vi "KeyboardSimulationCore.vi"(0 "Key Array":T3(array[cluster]) {"Key" items=["LBUTTON"=1, "RBUTTON"=2, "CANCEL"=3, "MBUTTON"=4, "BACKSPACE"=8, "TAB"=9, "CLEAR"=12, "ENTER"=13, "SHIFT"=16, "CTRL"=17, "ALT"=18, "PAUSE"=19, "CAPITAL"=20, "ESCAPE"=27, "SPACE"=32, "PAGEUP"=33, "PAGEDOWN"=34, "END"=35, "HOME"=36, "LEFTARROW"=37, "UPARROW"=38, "RIGHTARROW"=39, "DOWNARROW"=40, "SELECT"=41, "PRINT"=42, "EXECUTE"=43, "PRINTSCREEN"=44, "INSERT"=45, "DELETE"=46, "HELP"=47, "0"=48, "1"=49, "2"=50, "3"=51, "4"=52, "5"=53, "6"=54, "7"=55, "8"=56, "9"=57, "A"=65, "B"=66, "C"=67, "D"=68, "E"=69, "F"=70, "G"=71, "H"=72, "I"=73, "J"=74, "K"=75, "L"=76, "M"=77, "N"=78, "O"=79, "P"=80, "Q"=81, "R"=82, "S"=83, "T"=84, "U"=85, "V"=86, "W"=87, "X"=88, "Y"=89, "Z"=90, "LWIN"=91, "RWIN"=92, "APPS"=93, "NUMPAD0"=96, "NUMPAD1"=97, "NUMPAD2"=98, "NUMPAD3"=99, "NUMPAD4"=100, "NUMPAD5"=101, "NUMPAD6"=102, "NUMPAD7"=103, "NUMPAD8"=104, "NUMPAD9"=105, "MULTIPLY"=106, "ADD"=107, "SEPERATOR"=108, "SUBTRACT"=109, "DECIMAL"=110, "DIVIDE"=111, "F1"=112, "F2"=113, "F3"=114, "F4"=115, "F5"=116, "F6"=117, "F7"=118, "F8"=119, "F9"=120, "F10"=121, "F11"=122, "F12"=123, "F13"=124, "F14"=125, "F15"=126, "F16"=127, "F17"=128, "F18"=129, "F19"=130, "F20"=131, "F21"=132, "F22"=133, "F23"=134, "F24"=135, "NUMLOCK"=144, "SCROLL"=145, "LSHIFT"=160, "RSHIFT"=161, "LCTRL"=162, "RCTRL"=163, "LALT"=164, "RALT"=165, "VOLMUTE"=173, "VOLDOWN"=174, "VOLUP"=175, ";    :"=186, "=   +"=187, ",    <"=188, "-    _"=189, ".    >"=190, "/    ?"=191, "`    ~"=192, "[    {"=219, "\\    |"=220, "]    }"=221, "'    \""=222]}, 7 "Length of Key Press (ms)":u32=5, 11 "error in":errorcluster) -> (15 "error out":errorcluster)   [LabVIEW 2016, in "Drona.lvlib" / "KeyboardSimulation.lvlib"]
doc: "Handle the actions configured in the key array control for each of the configured keys"
uses:
  KeyboardSimulation.lvlib
  typedef/VirtualKey.ctl
  typedef/Action.ctl
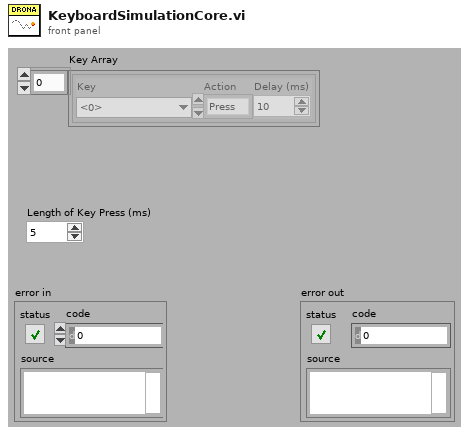
[diagram p1: front panel]
types:
  T1 = typedef "Drona.lvlib/KeyboardSimulation.lvlib/VirtualKey.ctl" = u8
  T2 = typedef "Drona.lvlib/KeyboardSimulation.lvlib/Action.ctl" = enum16{"Press", "Up", "Down"}
  T3 = cluster{"Key":T1, "Action":T2, "Delay (ms)":u32}[]
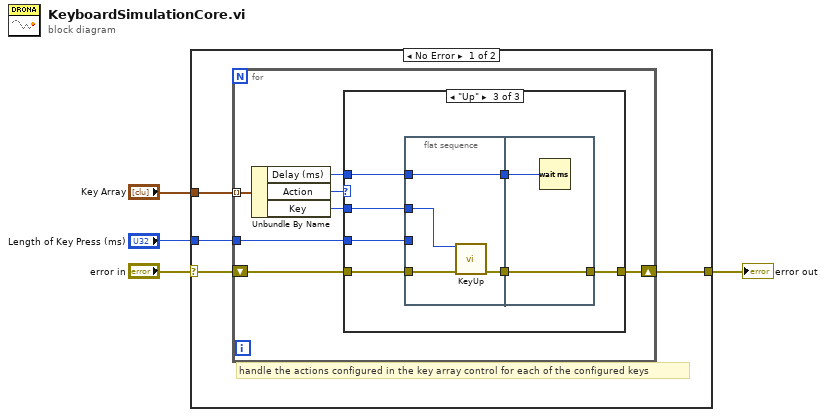
[diagram p0: block diagram]
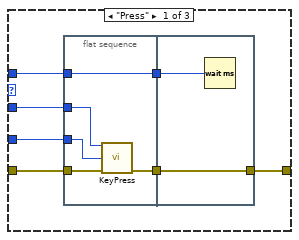
[diagram p2: hidden frame]
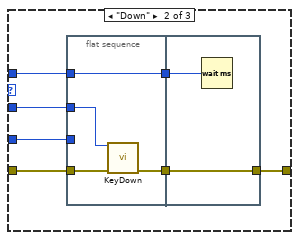
[diagram p3: hidden frame]
diagram:
  n1 = case shown="No Error" "error in" {
    selector: "error in" -> [w8 w56]
    tunnel: [w7 w56] -> w3
    tunnel: "Length of Key Press (ms)" -> [w6 _]
    tunnel: "Key Array" -> [w5 _]
    frame No Error {
      # "handle the actions configured in the key array control for each of the configured keys"
      n2 = for {
        tunnel: w5 -> [w15] mode=indexing
        tunnel: w6 -> [w14]
        shift-right: [w9] -> w7
        shift-left: w8 -> [w10]
        n3 = Unbundle By Name(w15) -> ("Delay (ms)"=w11:u32, "Action"=w13:T2, "Key"=w12:T1)
        n4 = case shown="\"Up\"" w13 {
          tunnel: w14 -> [w22 w36 w49]
          tunnel: w12 -> [w21 w35 w48]
          tunnel: w11 -> [w19 w33 w46]
          tunnel: w10 -> [w17 w31 w45]
          tunnel: [w16 w30 w43] -> w9
          frame "Press" {
            n5 = flat-sequence {
              tunnel: w22 -> [w24]
              tunnel: w21 -> [w23]
              tunnel: [w27] -> w20
              tunnel: w19 -> [w27]
              tunnel: [w25] -> w18
              tunnel: w17 -> [w26]
              tunnel: w20 -> [w29]
              tunnel: w18 -> [w28]
              tunnel: [w28] -> w16
              frame #0 {
                n6 = call "KeyPress.vi"("Virtual Key"=w23, "Millis"=w24, "error in"=w26) -> ("error out"=w25:errorcluster)  [unwired: 12 in]
              }
              frame #1 {
                n7 = Wait (ms)(milliseconds to wait=w29) -> ()  [unwired: 1 out]
              }
            }
          }
          frame "Down" {
            n8 = flat-sequence {
              tunnel: w36 -> [_]
              tunnel: w35 -> [w39]
              tunnel: [w40] -> w34
              tunnel: w33 -> [w40]
              tunnel: [w37] -> w32
              tunnel: w31 -> [w38]
              tunnel: w34 -> [w42]
              tunnel: w32 -> [w41]
              tunnel: [w41] -> w30
              frame #0 {
                n9 = call "KeyDown.vi"("Virtual Key"=w39, "error in"=w38) -> ("error out"=w37:errorcluster)  [unwired: 13 in]
              }
              frame #1 {
                n10 = Wait (ms)(milliseconds to wait=w42) -> ()  [unwired: 1 out]
              }
            }
          }
          frame "Up" {
            n11 = flat-sequence {
              tunnel: w49 -> [_]
              tunnel: w48 -> [w52]
              tunnel: [w53] -> w47
              tunnel: w46 -> [w53]
              tunnel: w45 -> [w51]
              tunnel: [w50] -> w44
              tunnel: w47 -> [w55]
              tunnel: w44 -> [w54]
              tunnel: [w54] -> w43
              frame #0 {
                n12 = call "KeyUp.vi"("Virtual Key"=w52, "error in"=w51) -> ("error out"=w50:errorcluster)  [unwired: 13 in]
              }
              frame #1 {
                n13 = Wait (ms)(milliseconds to wait=w55) -> ()  [unwired: 1 out]
              }
            }
          }
        }
      }
    }
    frame Error {
    }
  }
  "error out" <- w3
